vi "Update State.vi"(8 "error in (no error)":errorcluster, 10 "State":T1, 11 "Module in":refnum<class "Module.lvclass">) -> (0 "error out":errorcluster, 3 "Module out":refnum<class "Module.lvclass">)   [LabVIEW 2020, in "Volatus.lvlib" / "Module.lvclass"]
uses:
  Module.lvclass
  State.ctl
  Module.lvclass/Module.ctl
  Event Level.ctl
  Module Status Update.ctl
  MessageQ/MessageQ.lvclass/MessageQ.ctl
  MessageQ/MessageQ.lvclass
  Volatus.lvlib
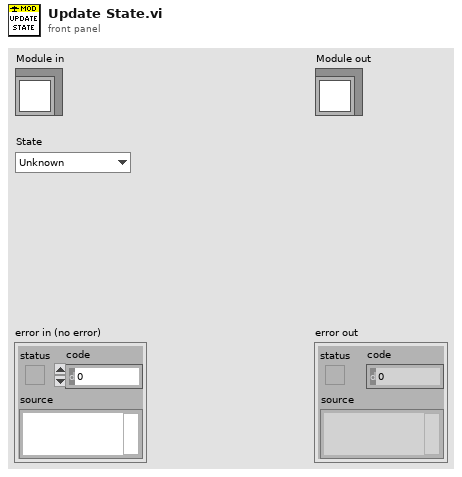
[diagram p1: front panel]
types:
  T1 = typedef "Volatus.lvlib/Module.lvclass/State.ctl" = enum16{"Unknown", "Launched", "Starting", "Running", "Stopping", "Stopped", "Error - Starting", "Error - Run", "Error - Stopping"}
  T2 = typedef "Volatus.lvlib/Event Level.ctl" = enum16{"Debug", "Info", "Warning", "Error"}
  T3 = typedef "Volatus.lvlib/Module Status Update.ctl" = cluster{"MessageQ":refnum<class "MessageQ.lvclass">, "State":T1, "Hierarchy":string[], "Forwarded":bool}
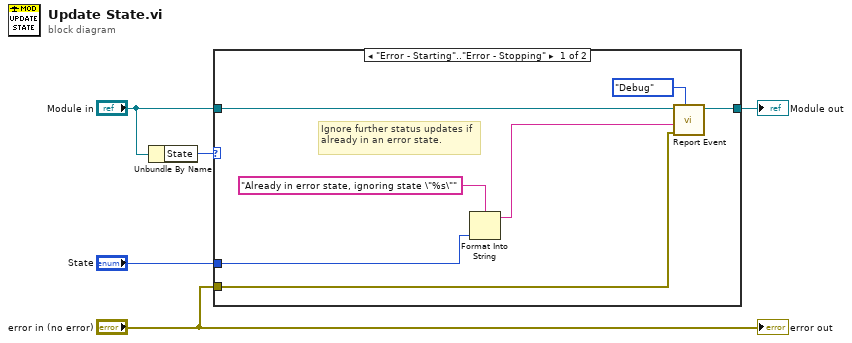
[diagram p0: block diagram]
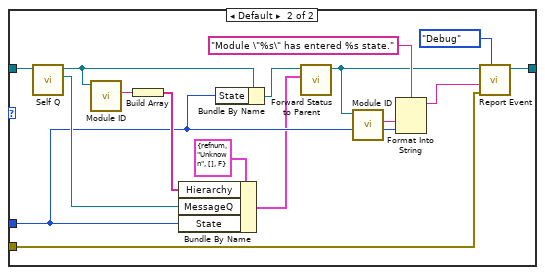
[diagram p2: hidden frame]
diagram:
  n1 = Unbundle By Name("Module in") -> ("State"=w2:T1)
  n2 = case shown="\"Error - Starting\"..\"Error - Stopping\"" w2 {
    tunnel: [w11 w26] -> w5
    tunnel: "State" -> [w7 w16]
    tunnel: "error in (no error)" -> [w6 w21]
    tunnel: "Module in" -> [w12 w17]
    frame "Error - Starting".."Error - Stopping" {
      # "Ignore further status updates if already in an error state."
      n3 = Format Into String(format string="Already in error state, ignoring state \"%s\"", w7) -> (resulting string=w8:string)  [unwired: 2 in, 1 out]
      n4 = call "Report Event.vi"("Level (Info)"=Event_Level."Debug", "error in (no error)"=w6, "Message"=w8, "Module in"=w12) -> ("Module out"=w11:refnum<class "Module.lvclass">)  [unwired: 6 in, 1 out]
    }
    frame Default {
      n5 = call "Self Q.vi"("Module in"=w17) -> ("Self Q"=w27:refnum<class "MessageQ.lvclass">, "Module out"=w20:refnum<class "Module.lvclass">)  [unwired: 9 in]
      n6 = call-dynamic "Module ID.vi"("Module in"=w20) -> ("Module ID"=w19:string)  [unwired: 10 in]
      n7 = Build Array(w19) -> (w18:string[])
      n8 = Bundle By Name(cluster=T3 {"MessageQ"=refnum, "State"=enum."Unknown", "Hierarchy"=[], "Forwarded"=FALSE} ("Nested State Data"), "Hierarchy"=w18, "MessageQ"=w27, "State"=w16) -> (w13:T3)
      n9 = Bundle By Name(cluster=w20, "State"=w16) -> (w15:refnum<class "Module.lvclass">)
      n10 = call "Forward Status to Parent.vi"("Module Status"=w13, "Module in"=w15) -> ("Module out"=w14:refnum<class "Module.lvclass">)  [unwired: 8 in, 1 out]
      n11 = call-dynamic "Module ID.vi"("Module in"=w14) -> ("Module ID"=w23:string)  [unwired: 10 in]
      n12 = Format Into String(format string="Module \"%s\" has entered %s state.", w23, w16) -> (resulting string=w22:string)  [unwired: 2 in, 1 out]
      n13 = call "Report Event.vi"("Level (Info)"=Event_Level."Debug", "error in (no error)"=w21, "Message"=w22, "Module in"=w14) -> ("Module out"=w26:refnum<class "Module.lvclass">)  [unwired: 6 in, 1 out]
    }
  }
  "Module out" <- w5
  "error out" <- "error in (no error)"
